vi "create stream from dataset.vi"(7 "fallback avro file (user documents\\nominal_fallback_files)":path, 11 "dataset":refnum<class "dataset.lvclass">) -> (0 "error out":errorcluster, 3 "stream session":refnum<data-value>)   [LabVIEW 2020, in "nominal core steps.lvlib"]
doc: "Create a reference to a stream to a provided dataset. Use `get dataset by rid` to get the dataset reference."
uses:
  nominal core steps.lvlib
  <vilib>/Nominal/Nominal IO Client/lv_src/datasources/dataset/dataset.lvclass
  stream session.ctl
  <vilib>/Nominal/Nominal IO Client/submodules/nominal-streaming-labview-ffi/lv_src/Stream/Stream.lvclass
  channel uid.ctl
  <vilib>/Nominal/Nominal IO Client/submodules/nominal-streaming-labview-ffi/lv_src/Channel/Channel.lvclass
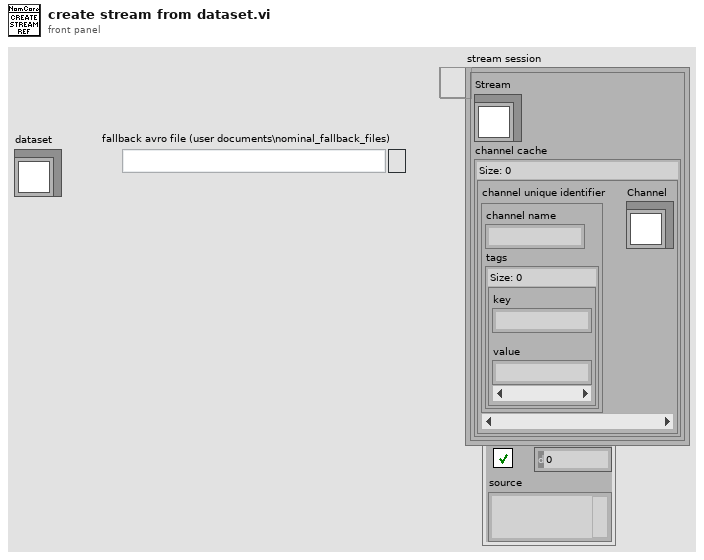
[diagram p1: front panel]
types:
  T1 = typedef "nominal core steps.lvlib/stream session.ctl" = cluster{"Stream":refnum<class "Stream.lvclass">, "channel cache":map{T2, refnum<class "Channel.lvclass">}}
  T2 = typedef "nominal core steps.lvlib/channel uid.ctl" = cluster{"channel name":string, "tags":map{string, string}}
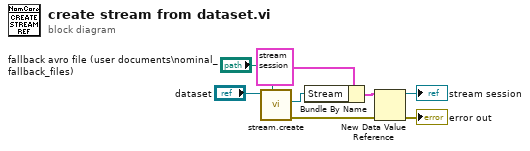
[diagram p0: block diagram]
diagram:
  n1 = call <vilib>:"stream.create.vi"("fallback avro file (user documents\\nominal_fallback_files)"="fallback avro file (user documents\\nominal_fallback_files)", "dataset in"="dataset") -> ("error out"=w7:errorcluster, "Stream"=w4:refnum<class "Stream.lvclass">)  [unwired: 7 in, 1 out]
  n2 = Bundle By Name(cluster=T1 {"Stream"=refnum, "channel cache"={}} ("stream session"), "Stream"=w4) -> (w3:T1)
  n3 = New Data Value Reference(data value=w3, error in=w7) -> (data value reference=→"stream session":refnum<data-value>, error out=→"error out":errorcluster)
